vi "Virtual DAQ Daten lesen und schreiben.vi"(8 "error in":errorcluster, 10 "Ausgabewerte":dbl[](array[numeric]), 11 "Auftrag":T1={"Messart"=enum."Wahl treffen", "Kanal"="", "PFI"="", "Rate"=1000.0, "Samples"=100, "Bereich"=10.0, "Kontinuierlich"=FALSE}) -> (0 "error out":errorcluster, 1 "Status":dbl, 2 "Signal":waveform(dbl)(graph), 3 "Daten":dbl[](array[numeric]))   [LabVIEW 2026]
doc: "Auftrag an die Steckwerkbank senden. Daten liefert die Messwerte. AO/DO verwenden Ausgabewerte. Der Widerstand steht in Daten[0] in Ohm."
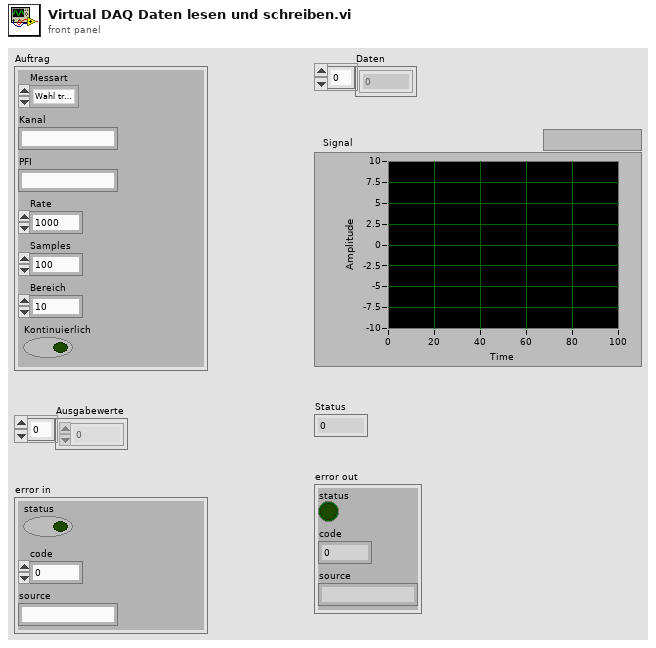
[diagram p1: front panel]
types:
  T1 = cluster{"Messart":enum8{"Wahl treffen", "AI Spannung", "AO Spannung", "DI Lesen", "DO Schreiben", "CTR Frequenz", "DMM Widerstand", "Ausgaenge freigeben"}, "Kanal":string, "PFI":string, "Rate":dbl, "Samples":i32, "Bereich":dbl, "Kontinuierlich":bool}
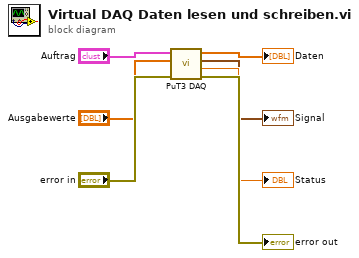
[diagram p0: block diagram]
diagram:
  n1 = call "PuT3 DAQ.vi"("error in"="error in", "Ausgabewerte"="Ausgabewerte", "Auftrag"="Auftrag") -> ("error out"=→"error out":errorcluster, "Status"=→"Status":dbl, "Signal"=→"Signal":waveform(dbl), "Daten"=→"Daten":dbl[])  [unwired: 5 in]
